vi "subtract-separate.vi"() -> ()   [LabVIEW 2026]
panel:
  out "result":i32
  in  "y":i32
  in  "x":i32
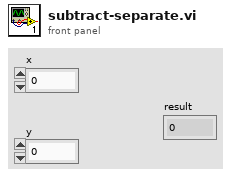
[diagram p1: front panel]
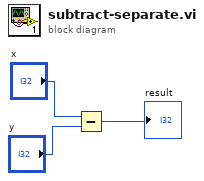
[diagram p0: block diagram]
diagram:
  n1 = Subtract(x="x", y="y") -> (x-y=→"result":i32)
